vi "AppendInspectionRow.vi"(6 "error in (no error)":errorcluster, 8 "Row":string, 9 "FilePath":path) -> (0 "error out":errorcluster)   [LabVIEW 2026]
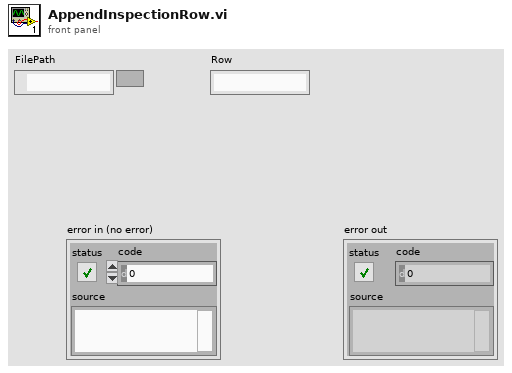
[diagram p1: front panel]
types:
  T1 = enum16{"open", "replace", "create", "open or create", "replace or create", "replace or create with confirmation"}
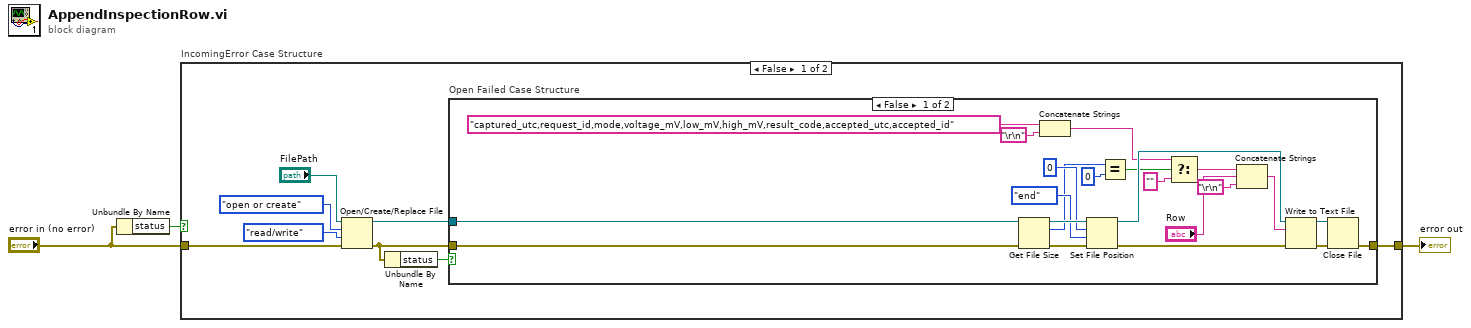
[diagram p0: block diagram]
diagram:
  n1 = Unbundle By Name("error in (no error)") -> ("status"=w3:bool)
  n2 = case "IncomingError Case Structure" shown="False" w3 {
    tunnel: [w5 w35] -> w2
    tunnel: "error in (no error)" -> [w10 w35]
    frame False {
      n3 = Open/Create/Replace File(file path (use dialog)="FilePath", error in=w10, operation (0:open)=T1."open or create", access (0:read/write)=enum16{"read/write", "read-only", "write-only"}."read/write") -> (refnum out=w4:refnum<file>, error out=w6:errorcluster)  [unwired: 2 in, 1 out]
      n4 = Unbundle By Name(w6) -> ("status"=w7:bool)
      n5 = case "Open Failed Case Structure" shown="False" w7 {
        tunnel: w6 -> [w33 w34]
        tunnel: [w29 w34] -> w5
        tunnel: w4 -> [w28 _]
        frame False {
          n6 = Get File Size(file=w28, error in=w33) -> (refnum out=w27:refnum<file>, size (in bytes)=w22:i64, 0:w32:errorcluster)
          n7 = Concatenate Strings("captured_utc,request_id,mode,voltage_mV,low_mV,high_mV,result_code,accepted_utc,accepted_id" ("text"), "\r\n") -> (w18:string)
          n8 = Set File Position(offset (in bytes) (0)=i64 0, refnum=w27, from (0:start)=enum16{"start", "end", "current"}."end", error in=w32) -> (refnum out=w24:refnum<file>, error out=w31:errorcluster)
          n9 = Equal?(x=w22, y=i64 0) -> (x = y?=w17:bool)
          n10 = Select(t=w18, s=w17, f="") -> (s? t:f=w15:string)
          n11 = Concatenate Strings(w15, "Row", "\r\n") -> (w12:string)
          n12 = Write to Text File(file (use dialog)=w24, text=w12, error in=w31) -> (refnum out=w23:refnum<file>, error out=w30:errorcluster)  [unwired: 1 in, 1 out]
          n13 = Close File(refnum=w23, error in=w30) -> (error out=w29:errorcluster)  [unwired: 1 out]
        }
        frame True {
        }
      }
    }
    frame True {
    }
  }
  "error out" <- w2
